vi "_lcod_CFX_data.vi"(8 "error in":errorcluster caption="错误输入", 10 "data":string[][](table), 11 "CFX":T1) -> (0 "error out":errorcluster caption="错误输出", 3 "CfxData":T3)   [LabVIEW 2025]
uses:
  ctl/CFX_data.ctl
  ctl/CFX_trigger.ctl
  ctl/CfxTopic-cmd.ctl
  <vilib>/Utility/error.llb/Trim Whitespace One-Sided.vi
  <vilib>/regexp/Match Regular Expression.xnode
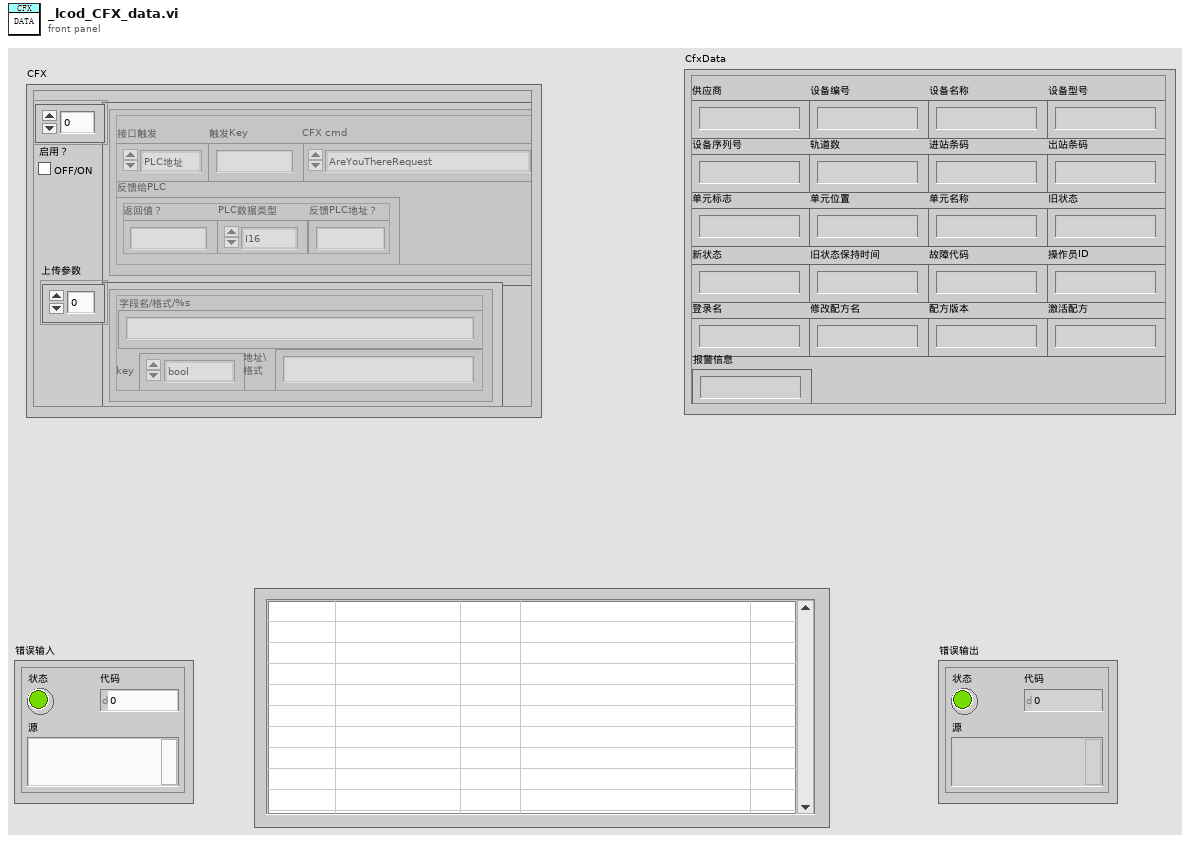
[diagram p1: front panel]
types:
  T1 = typedef "CFX_trigger.ctl" = cluster{"CFX":cluster{"URL trigger":enum16{"PLC地址", "值改变", "time", "Bool[]", "alarm"}, "trigger Key":string, "CFX cmd":T2, "InPlc":cluster{"Out OK?":string, "PlcDadtKye":enum16{"I16", "Bool", "Ascll"}, "Plc_Address":string}}[], "Enable?":bool, "Upload":cluster{"name":string, "key":enum16{"bool", "str", "value", "time", "alarm", "i32>str[]", "Ascll", "str>offse"}, "address":string}[]}
  T2 = typedef "CfxTopic-cmd.ctl" = enum16{"AreYouThereRequest", "AreYouThereResponse", "EndpointConnected", "EndpointShuttingDown", "GetEndpointInformationRequest", "GetEndpointInformationResponse", "Heartbeat", "NotSupportedResponse", "WhoIsThereRequest", "WhoIsThereResponse", "UnitArrived", "UnitsDeparted", "StationStateChanged", "FaultOccurred", "FaultCleared", "OperatorActivated", "OperatorDeactivated", "RecipeModified", "RecipeActived", "ActivateRecipeRequest", "ActivateRecipeResponse"}
  T3 = typedef "CFX_data.ctl" = cluster{"Vendor":string, "UniqueIdentifier":string, "FriendlyName":string, "ModelNumber":string, "SerialNumber":string, "NumberofLanes":string, "CodeIn":string, "CodeOut":string, "Unitldentifer":string, "PositionNumber":string, "PositionName":string, "OldState":string, "NewState":string, "OldStateDuration":string, "Faultcode":string, "Operatorldentifer":string, "LoginName":string, "RecipeName":string, "Revision":string, "Activate formula":string, "Description":string}
  T4 = cluster{"name":string, "key":enum16{"bool", "str", "value", "time", "alarm", "i32>str[]", "Ascll", "str>offse"}, "address":string}[]
  T5 = enum16{"bool", "str", "value", "time", "alarm", "i32>str[]", "Ascll", "str>offse"}
  T6 = cluster{"[0]":string, "[1]":string, "[2]":string, "[3]":string, "[4]":string, "[5]":string, "[6]":string, "[7]":string, "[8]":string, "[9]":string, "[10]":string, "[11]":string, "[12]":string, "[13]":string, "[14]":string, "[15]":string, "[16]":string, "[17]":string, "[18]":string, "[19]":string, "[20]":string}
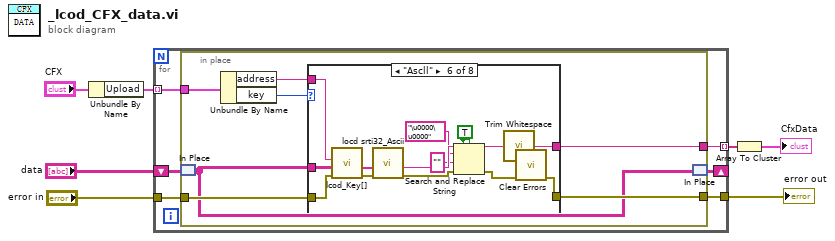
[diagram p0: block diagram]
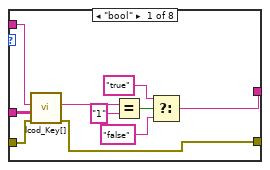
[diagram p2: hidden frame]
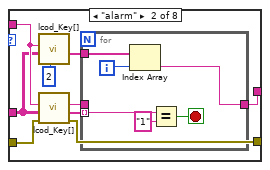
[diagram p3: hidden frame]
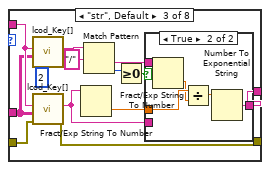
[diagram p4: hidden frame]
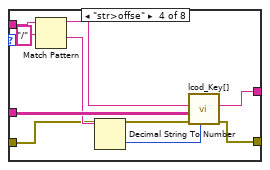
[diagram p6: hidden frame]
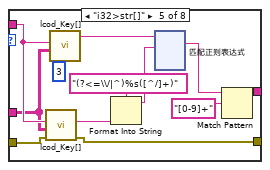
[diagram p7: hidden frame]
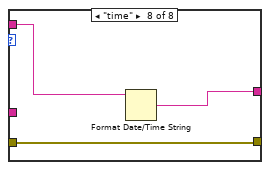
[diagram p9: hidden frame]
diagram:
  n1 = Unbundle By Name("CFX") -> ("Upload"=w7:T4)
  n2 = for {
    tunnel: "error in" -> [w13]
    tunnel: [w12] -> w5
    tunnel: w7 -> [w11] mode=indexing
    shift-right: [w9] -> _
    shift-left: "data" -> [w10]
    tunnel: [w8] -> w3 mode=indexing
    n3 = in-place {
      in-place-border: w13 -> [w18]
      in-place-border: [w17] -> w12
      in-place-border: w11 -> [w16]
      in-place-border: [w14] -> w8
      n4 = in-place-match #1(w10) -> (w15:string[][])
      n5 = Unbundle By Name(w16) -> ("address"=w20:string, "key"=w19:T5)
      n6 = case shown="\"Ascll\"" w19 {
        tunnel: w20 -> [w24 w36 w58 w71 w84 w215 w218 w221]
        tunnel: w15 -> [w25 w33 w57 w73 w76 w216 _ _]
        tunnel: [w23 w39 w49 w67 w78 w210 w218 w220] -> w14
        tunnel: w18 -> [w22 w32 w47 w66 w75 w204 w217 w219]
        tunnel: [w21 w31 w46 w65 w74 w203 w217 w219] -> w17
        frame "bool" {
          n7 = call "lcod_Key[].vi"("Error In"=w22, "PLC data"=w25, "key in"=w24) -> ("Error Out"=w21:errorcluster, "value"=w30:string)  [unwired: 6 in, 1 out]
          n8 = Equal?(x=w30, y="1") -> (x = y?=w28:bool)
          n9 = Select(t="true" ("y"), s=w28, f="false" ("y")) -> (s? t:f=w23:string)
        }
        frame "alarm" {
          n10 = call "lcod_Key[].vi"("index"=2, "PLC data"=w33, "key in"=w36) -> ("value[]"=w34:string[])  [unwired: 6 in, 2 out]
          n11 = call "lcod_Key[].vi"("Error In"=w32, "PLC data"=w33, "key in"=w36) -> ("Error Out"=w31:errorcluster, "value[]"=w38:string[], "value"=w37:string)  [unwired: 6 in]
          n12 = for {
            tunnel: w38 -> [w45] mode=indexing
            tunnel: [w40] -> w39
            tunnel: w37 -> [_]
            tunnel: w34 -> [w42]
            i -> [w41]
            stop <- w43 stop-if-true
            n13 = Index Array(array=w42, index=w41) -> (element=w40:string)
            n14 = Equal?(x=w45, y="1") -> (x = y?=w43:bool)
          }
        }
        frame "str", Default {
          n15 = call "lcod_Key[].vi"("index"=2, "PLC data"=w57, "key in"=w58) -> ("value"=w55:string)  [unwired: 6 in, 2 out]
          n16 = call "lcod_Key[].vi"("Error In"=w47, "PLC data"=w57, "key in"=w58) -> ("Error Out"=w46:errorcluster, "value"=w48:string)  [unwired: 6 in, 1 out]
          n17 = Fract/Exp String To Number(string=w48) -> (number=w50:dbl)  [unwired: 3 in, 1 out]
          n18 = Match Pattern(string=w55, regular expression="/" ("正则表达式")) -> (after substring=w51:string, offset past match=w53:i32)  [unwired: 1 in, 2 out]
          n19 = Greater Or Equal To 0?(x=w53) -> (x >= 0?=w52:bool)
          n20 = case shown="True" w52 {
            tunnel: w51 -> [_ w64]
            tunnel: w50 -> [_ w63]
            tunnel: [w59 w60] -> w49
            tunnel: w48 -> [w59 _]
            frame False {
            }
            frame True {
              n21 = Fract/Exp String To Number(string=w64) -> (number=w62:dbl)  [unwired: 3 in, 1 out]
              n22 = Divide(x=w63, y=w62) -> (x/y=w61:dbl)
              n23 = Number To Exponential String(number=w61) -> (E-format string=w60:string)  [unwired: 3 in]
            }
          }
        }
        frame "str>offse" {
          n24 = Match Pattern(string=w71, regular expression="/" ("正则表达式")) -> (before substring=w70:string, after substring=w68:string)  [unwired: 1 in, 2 out]
          n25 = Decimal String To Number(string=w68) -> (number=w69:i32)  [unwired: 2 in, 1 out]
          n26 = call "lcod_Key[].vi"("index"=w69, "Error In"=w66, "PLC data"=w73, "key in"=w70) -> ("Error Out"=w65:errorcluster, "value"=w67:string)  [unwired: 5 in, 1 out]
        }
        frame "i32>str[]" {
          n27 = call "lcod_Key[].vi"("Error In"=w75, "PLC data"=w76, "key in"=w84) -> ("Error Out"=w74:errorcluster, "value"=w82:string)  [unwired: 6 in, 1 out]
          n28 = call "lcod_Key[].vi"("index"=3, "PLC data"=w76, "key in"=w84) -> ("value"=w83:string)  [unwired: 6 in, 2 out]
          n29 = Format Into String(format string="(?<=\\/|^)%s([^/]+)" ("正则表达式"), w82) -> (resulting string=w81:string)  [unwired: 2 in, 1 out]
          n30 = xnode "匹配正则表达式"("输入字符串"=w83, "正则表达式"=w81) -> ("所有匹配"=w79:string)  [unwired: 4 in, 4 out]
          n31 = Match Pattern(string=w79, regular expression="[0-9]+" ("正则表达式")) -> (after substring=w78:string)  [unwired: 1 in, 3 out]
        }
        frame "Ascll" {
          w205 = TRUE ("替换全部？(F)")
          n32 = call "lcod_Key[].vi"("Error In"=w204, "PLC data"=w216, "key in"=w215) -> ("Error Out"=w213:errorcluster, "value[]"=w214:string[])  [unwired: 6 in, 1 out]
          n33 = call "locd srti32_Ascii.vi"("Error In"=w213, "in stri32"=w214) -> ("Error Out"=w209:errorcluster, "i6_str"=w211:string)  [unwired: 8 in]
          n34 = Search and Replace String(replace all?=w205, case sensitive?=w205, input string=w211, search string="\u0000\u0000" ("搜索字符串"), replace string="" ("替换字符串(\"\")"), error in=w209) -> (result string=w212:string, error out=w208:errorcluster)  [unwired: 2 in, 2 out]
          n35 = call <vilib>:"Trim Whitespace.vi"("string"=w212) -> ("trimmed string"=w210:string)  [unwired: 1 in]
          n36 = call <vilib>:"Clear Errors.vi"("error in (no error)"=w208) -> ("error out"=w203:errorcluster)  [unwired: 5 in, 1 out]
        }
        frame "value" {
        }
        frame "time" {
          n37 = Format Date/Time String(time format string (%c)=w221) -> (date/time string=w220:string)  [unwired: 2 in]
        }
      }
      n38 = in-place-match #1(w15) -> (w9:string[][])
    }
  }
  "error out" <- w5
  n39 = Array To Cluster(array=w3) -> (cluster=→"CfxData":T6)
